vi "ASD Signal SE caluculation VI.vi"(7 "1s datapoint":i32, 8 "Region Start":i32, 9 "RS End":i32[](array[numeric]), 10 "RS Start":i32[](array[numeric]), 11 "R Peak location":i32[](array[numeric])) -> (0 "Signal Time (ms)":dbl[](array[numeric]), 1 "T END Time (s)":dbl[](array[numeric]), 2 "T Start Time (s)":dbl[](array[numeric]), 3 "TS Peak Time (s)":dbl[](array[numeric]))   [LabVIEW 2018]
panel:
  out "x/y 2":dbl
  out "x/y":dbl
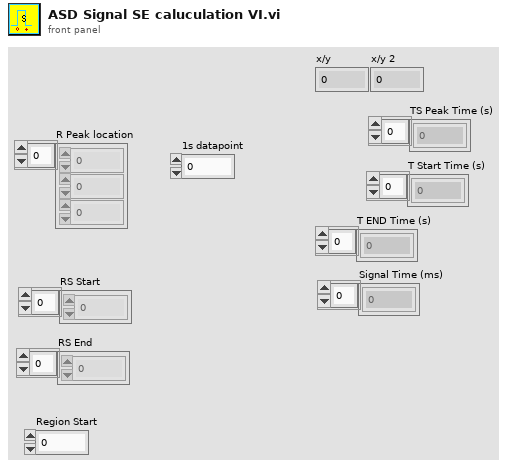
[diagram p1: front panel]
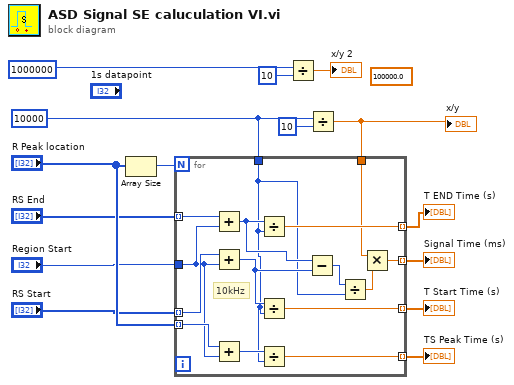
[diagram p0: block diagram]
diagram:
  (unwired) 100000.0 ("x")
  w6 = 10000 ("y")
  n1 = Array Size(array="R Peak location") -> (size(s)=w15:i32)
  n2 = Divide(x=1000000 ("y"), y=10) -> (x/y=→"x/y 2":dbl)
  n3 = Divide(x=w6, y=10) -> (x/y=w4:dbl)
  "x/y" <- w4
  n4 = for {
    N: w15 -> [_]
    tunnel: "R Peak location" -> [w30] mode=indexing
    tunnel: "Region Start" -> [w27]
    tunnel: "RS Start" -> [w29] mode=indexing
    tunnel: "RS End" -> [w28] mode=indexing
    tunnel: [w25] -> w10 mode=indexing
    tunnel: [w23] -> w9 mode=indexing
    tunnel: [w24] -> w8 mode=indexing
    tunnel: [w22] -> w7 mode=indexing
    tunnel: w6 -> [w17]
    tunnel: w4 -> [w16]
    # "10kHz"
    n5 = Add(x=w28, y=w27) -> (x+y=w21:i32)
    n6 = Add(x=w29, y=w27) -> (x+y=w20:i32)
    n7 = Add(x=w30, y=w27) -> (x+y=w26:i32)
    n8 = Divide(x=w21, y=w17) -> (x/y=w24:dbl)
    n9 = Divide(x=w20, y=w17) -> (x/y=w23:dbl)
    n10 = Divide(x=w26, y=w17) -> (x/y=w25:dbl)
    n11 = Subtract(x=w21, y=w20) -> (x-y=w19:i32)
    n12 = Divide(x=w19, y=w17) -> (x/y=w18:dbl)
    n13 = Multiply(x=w16, y=w18) -> (x*y=w22:dbl)
  }
  "TS Peak Time (s)" <- w10
  "T Start Time (s)" <- w9
  "T END Time (s)" <- w8
  "Signal Time (ms)" <- w7
